vi "HID_READ.vi"() -> ()   [LabVIEW 2017]
uses:
  <userlib>/HID_ARZ/HID_ARZ.lvlib
panel:
  out "led2":bool
  out "led1":bool
  out "Meter":dbl(knob) scale=0.0..5.0
  out "Thermometer":dbl(slide) scale=0.0..100.0
  out "string":string
  out "Conectado":bool
  in  "stop":bool
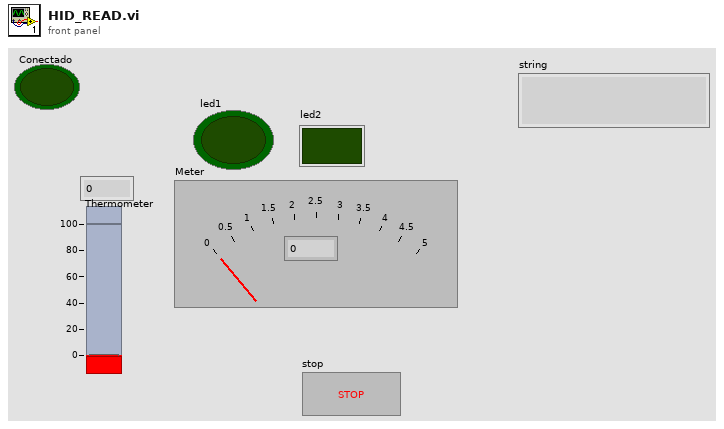
[diagram p1: front panel]
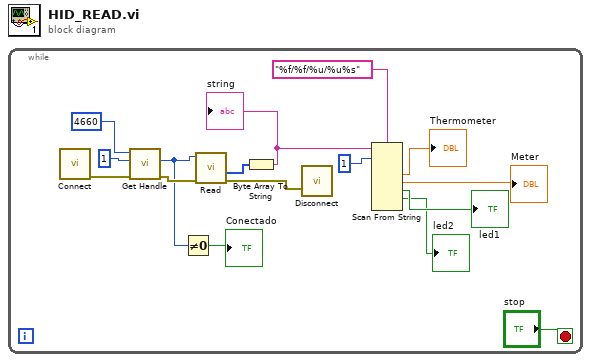
[diagram p0: block diagram]
diagram:
  n1 = while {
    stop <- "stop" stop-if-true
    n2 = call <userlib>:"Connect.vi"() -> ("error out"=w15:errorcluster)  [unwired: 9 in, 2 out]
    n3 = call <userlib>:"Get Handle.vi"("error in (no error)"=w15, "PID"=u32 1, "VID"=u32 4660) -> ("error out"=w11:errorcluster, "HANDLE"=w10:u32)  [unwired: 7 in]
    n4 = Not Equal To 0?(x=w10) -> (x != 0?=→"Conectado":bool)
    n5 = call <userlib>:"Read.vi"("error in (no error)"=w11, "HANDLE"=w10) -> ("error out"=w8:errorcluster, "BUFFER"=w9:u8[])  [unwired: 7 in, 1 out]
    n6 = Byte Array To String(unsigned byte array=w9) -> (string=w7:string)
    "string" <- w7
    n7 = call <userlib>:"Disconnect.vi"("error in (no error)"=w8) -> ()  [unwired: 10 in, 1 out]
    n8 = Scan From String(format string="%f/%f/%u/%u%s", input string=w7, initial scan location=u32 1) -> (output 1=→"Thermometer":dbl, output 2=→"Meter":dbl, output 3=→"led1":bool, output 4=→"led2":bool)  [unwired: 7 in, 3 out]
  }
